vi "Abstract LV Class - Hierarchy.vi"   [LabVIEW 2021]
uses:
  Type/Abs_Type.lvclass
  Value/Abs_Value.lvclass
  Numeric/Abs_Numeric.lvclass
  Floating Point/Abs_Floating Point.lvclass
  Single Float/Abs_Single Float.lvclass
  Double Float/Abs_Double Float.lvclass
  Extended Float/Abs_Extended Float.lvclass
  Complex Double Float/Abs_Complex Double Float.lvclass
  Complex Extended Float/Abs_Complex Extended Float.lvclass
  Complex Single Float/Abs_Complex Single Float.lvclass
  Integer/Abs_Integer.lvclass
  I8 Integer/Abs_I8 Integer.lvclass
  I16 Integer/Abs_I16 Integer.lvclass
  I32 Integer/Abs_I32 Integer.lvclass
  I64 Integer/Abs_I64 Integer.lvclass
  U8 Integer/Abs_U8 Integer.lvclass
  U16 Integer/Abs_U16 Integer.lvclass
  U32 Integer/Abs_U32 Integer.lvclass
  U64 Integer/Abs_U64 Integer.lvclass
  Time/Abs_Time.lvclass
  Boolean/Abs_Boolean.lvclass
  String/Abs_String.lvclass
  Variant/Abs_Variant.lvclass
  Waveform/Abs_Waveform.lvclass
  Boolean/Static Write.vi
  Double Float/Simple Read.vi
  Boolean/Static Read.vi
panel:
  # "SEE DIAGRAM\nFOR Hierarchy"
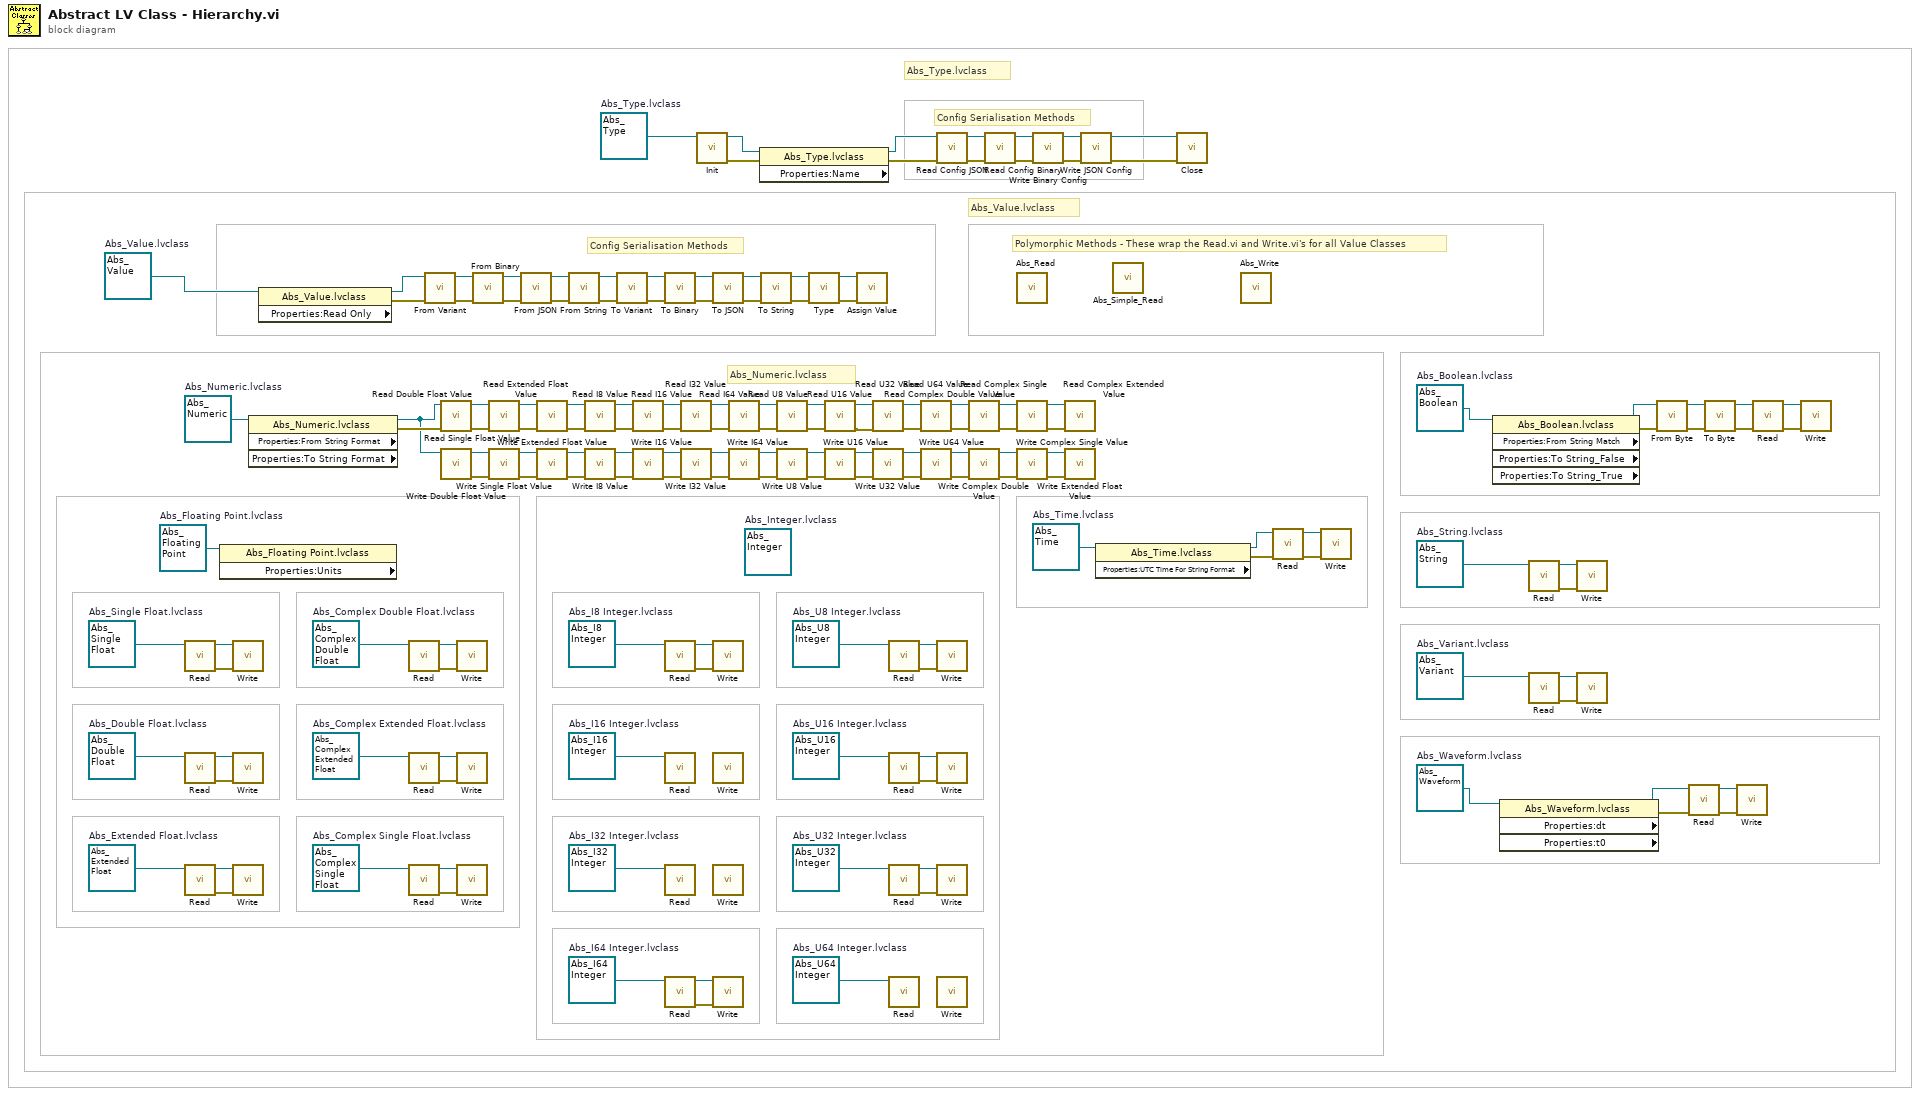
[diagram p0: block diagram]
diagram:
  w43 = refnum<class "Abs_Waveform.lvclass"> refnum  # Abs_Waveform.lvclass
  w44 = refnum<class "Abs_Variant.lvclass"> refnum  # Abs_Variant.lvclass
  w49 = refnum<class "Abs_String.lvclass"> refnum  # Abs_String.lvclass
  w58 = refnum<class "Abs_Boolean.lvclass"> refnum  # Abs_Boolean.lvclass
  w63 = refnum<class "Abs_Time.lvclass"> refnum  # Abs_Time.lvclass
  w73 = refnum<class "Abs_U64 Integer.lvclass"> refnum  # Abs_U64 Integer.lvclass
  w72 = refnum<class "Abs_U32 Integer.lvclass"> refnum  # Abs_U32 Integer.lvclass
  w70 = refnum<class "Abs_U16 Integer.lvclass"> refnum  # Abs_U16 Integer.lvclass
  w71 = refnum<class "Abs_U8 Integer.lvclass"> refnum  # Abs_U8 Integer.lvclass
  w76 = refnum<class "Abs_I64 Integer.lvclass"> refnum  # Abs_I64 Integer.lvclass
  w75 = refnum<class "Abs_I32 Integer.lvclass"> refnum  # Abs_I32 Integer.lvclass
  w74 = refnum<class "Abs_I16 Integer.lvclass"> refnum  # Abs_I16 Integer.lvclass
  w81 = refnum<class "Abs_I8 Integer.lvclass"> refnum  # Abs_I8 Integer.lvclass
  (unwired) refnum<class "Abs_Integer.lvclass"> refnum  # Abs_Integer.lvclass
  w84 = refnum<class "Abs_Complex Single Float.lvclass"> refnum  # Abs_Complex Single Float.lvclass
  w87 = refnum<class "Abs_Complex Extended Float.lvclass"> refnum  # Abs_Complex Extended Float.lvclass
  w90 = refnum<class "Abs_Complex Double Float.lvclass"> refnum  # Abs_Complex Double Float.lvclass
  w93 = refnum<class "Abs_Extended Float.lvclass"> refnum  # Abs_Extended Float.lvclass
  w96 = refnum<class "Abs_Double Float.lvclass"> refnum  # Abs_Double Float.lvclass
  w99 = refnum<class "Abs_Single Float.lvclass"> refnum  # Abs_Single Float.lvclass
  w100 = refnum<class "Abs_Floating Point.lvclass"> refnum  # Abs_Floating Point.lvclass
  w128 = refnum<class "Abs_Numeric.lvclass"> refnum  # Abs_Numeric.lvclass
  w38 = refnum<class "Abs_Value.lvclass"> refnum  # Abs_Value.lvclass
  w151 = refnum<class "Abs_Type.lvclass"> refnum  # Abs_Type.lvclass
  # "Abs_Numeric.lvclass"
  # "Polymorphic Methods - These wrap the Read.vi and Write.vi's for all Value Classes"
  # "Config Serialisation Methods"
  # "Abs_Value.lvclass"
  # "Abs_Type.lvclass"
  # "Config Serialisation Methods"
  n1 = call-dynamic "Read.vi"("Double Float.lvclass_340760 in"=w99) -> ("error out"=w97:errorcluster, "Double Float.lvclass_340760 out"=w98:refnum<class "Abs_Single Float.lvclass">)  [unwired: 8 in, 1 out]
  n2 = call-dynamic "Read.vi"("Double Float.lvclass_340760 in"=w96) -> ("error out"=w94:errorcluster, "Double Float.lvclass_340760 out"=w95:refnum<class "Abs_Double Float.lvclass">)  [unwired: 8 in, 1 out]
  n3 = call-dynamic "Read.vi"("Double Float.lvclass_340760 in"=w93) -> ("error out"=w91:errorcluster, "Double Float.lvclass_340760 out"=w92:refnum<class "Abs_Extended Float.lvclass">)  [unwired: 8 in, 1 out]
  n4 = property class="Abs_Floating Point.lvclass" props=["Properties:Units"](reference=w100) -> ()  [unwired: 1 in, 3 out]
  n5 = call-dynamic "Write.vi"("error in (no error)"=w97, "Double Float.lvclass_340760 in"=w98) -> ()  [unwired: 8 in, 2 out]
  n6 = call-dynamic "Write.vi"("error in (no error)"=w94, "Double Float.lvclass in"=w95) -> ()  [unwired: 8 in, 2 out]
  n7 = call-dynamic "Write.vi"("error in (no error)"=w91, "Double Float.lvclass_340760 in"=w92) -> ()  [unwired: 8 in, 2 out]
  n8 = property class="Abs_Numeric.lvclass" props=["Properties:From String Format", "Properties:To String Format"](reference=w128) -> (reference out=w29:refnum<class "Abs_Numeric.lvclass">, error out=w127:errorcluster)  [unwired: 1 in, 2 out]
  n9 = property class="Abs_Value.lvclass" props=["Properties:Read Only"](reference=w38) -> (reference out=w36:refnum<class "Abs_Value.lvclass">, error out=w37:errorcluster)  [unwired: 1 in, 1 out]
  n10 = call-dynamic "Read.vi"("Double Float.lvclass_340760 in"=w90) -> ("error out"=w88:errorcluster, "Double Float.lvclass_340760 out"=w89:refnum<class "Abs_Complex Double Float.lvclass">)  [unwired: 8 in, 1 out]
  n11 = call-dynamic "Read.vi"("Double Float.lvclass_340760 in"=w87) -> ("error out"=w85:errorcluster, "Double Float.lvclass_340760 out"=w86:refnum<class "Abs_Complex Extended Float.lvclass">)  [unwired: 8 in, 1 out]
  n12 = call-dynamic "Read.vi"("Double Float.lvclass_340760 in"=w84) -> ("error out"=w82:errorcluster, "Double Float.lvclass_340760 out"=w83:refnum<class "Abs_Complex Single Float.lvclass">)  [unwired: 8 in, 1 out]
  n13 = call-dynamic "From Variant.vi"("error in (no error)"=w37, "Abs_Value in"=w36) -> ("error out"=w34:errorcluster, "Abs_Value out"=w35:refnum<class "Abs_Value.lvclass">)  [unwired: 8 in]
  n14 = call-dynamic "Read Double Float Value.vi"("error in (no error)"=w127, "Numeric in"=w29) -> ("error out"=w117:errorcluster, "Numeric out"=w126:refnum<class "Abs_Numeric.lvclass">)  [unwired: 7 in, 1 out]
  n15 = call-dynamic "Write Double Float Value.vi"("Numeric in"=w29) -> ("error out"=w15:errorcluster, "Numeric out"=w28:refnum<class "Abs_Numeric.lvclass">)  [unwired: 9 in]
  n16 = call-dynamic "Write.vi"("error in (no error)"=w88, "Double Float.lvclass_340760 in"=w89) -> ()  [unwired: 8 in, 2 out]
  n17 = call-dynamic "Write.vi"("error in (no error)"=w85, "Double Float.lvclass_340760 in"=w86) -> ()  [unwired: 8 in, 2 out]
  n18 = call-dynamic "Write.vi"("error in (no error)"=w82, "Double Float.lvclass_340760 in"=w83) -> ()  [unwired: 8 in, 2 out]
  n19 = call-dynamic "From Binary.vi"("error in (no error)"=w34, "Type in"=w35) -> ("error out"=w133:errorcluster, "Type out"=w138:refnum<class "Abs_Value.lvclass">)  [unwired: 7 in, 1 out]
  n20 = call-dynamic "Read Single Float Value.vi"("error in (no error)"=w117, "Numeric in"=w126) -> ("error out"=w116:errorcluster, "Numeric out"=w125:refnum<class "Abs_Numeric.lvclass">)  [unwired: 7 in, 1 out]
  n21 = call-dynamic "Write Single Float Value.vi"("error in (no error)"=w15, "Numeric in"=w28) -> ("error out"=w14:errorcluster, "Numeric out"=w27:refnum<class "Abs_Numeric.lvclass">)  [unwired: 8 in]
  n22 = call-dynamic "From JSON.vi"("error in (no error)"=w133, "Type in"=w138) -> ("error out"=w132:errorcluster, "Type out"=w137:refnum<class "Abs_Value.lvclass">)  [unwired: 8 in]
  n23 = call-dynamic "Read Extended Float Value.vi"("error in (no error)"=w116, "Numeric in"=w125) -> ("error out"=w115:errorcluster, "Numeric out"=w124:refnum<class "Abs_Numeric.lvclass">)  [unwired: 7 in, 1 out]
  n24 = call-dynamic "Write Extended Float Value.vi"("error in (no error)"=w14, "Numeric in"=w27) -> ("error out"=w13:errorcluster, "Numeric out"=w26:refnum<class "Abs_Numeric.lvclass">)  [unwired: 8 in]
  n25 = call-dynamic "From String.vi"("error in (no error)"=w132, "Type in"=w137) -> ("error out"=w32:errorcluster, "Type out"=w33:refnum<class "Abs_Value.lvclass">)  [unwired: 6 in, 2 out]
  n26 = call-dynamic "Read I8 Value.vi"("error in (no error)"=w115, "Numeric in"=w124) -> ("error out"=w114:errorcluster, "Numeric out"=w123:refnum<class "Abs_Numeric.lvclass">)  [unwired: 7 in, 1 out]
  n27 = call-dynamic "Write I8 Value.vi"("error in (no error)"=w13, "Numeric in"=w26) -> ("error out"=w12:errorcluster, "Numeric out"=w25:refnum<class "Abs_Numeric.lvclass">)  [unwired: 8 in]
  n28 = call-dynamic "To Variant.vi"("error in (no error)"=w32, "Abs_Value in"=w33) -> ("error out"=w30:errorcluster, "Abs_Value out"=w31:refnum<class "Abs_Value.lvclass">)  [unwired: 7 in, 1 out]
  n29 = call-dynamic "Read I16 Value.vi"("error in (no error)"=w114, "Numeric in"=w123) -> ("error out"=w113:errorcluster, "Numeric out"=w122:refnum<class "Abs_Numeric.lvclass">)  [unwired: 7 in, 1 out]
  n30 = call-dynamic "Write I16 Value.vi"("error in (no error)"=w12, "Numeric in"=w25) -> ("error out"=w11:errorcluster, "Numeric out"=w24:refnum<class "Abs_Numeric.lvclass">)  [unwired: 8 in]
  n31 = call-dynamic "To Binary.vi"("error in (no error)"=w30, "Type in"=w31) -> ("error out"=w131:errorcluster, "Type out"=w136:refnum<class "Abs_Value.lvclass">)  [unwired: 7 in, 1 out]
  n32 = call-dynamic "Read.vi"("Double Float.lvclass_340760 in"=w81) -> ("error out"=w79:errorcluster, "Double Float.lvclass_340760 out"=w80:refnum<class "Abs_I8 Integer.lvclass">)  [unwired: 8 in, 1 out]
  n33 = call-dynamic "Read.vi"("Double Float.lvclass_340760 in"=w74) -> ()  [unwired: 8 in, 3 out]
  n34 = call-dynamic "Read.vi"("Double Float.lvclass_340760 in"=w75) -> ()  [unwired: 8 in, 3 out]
  n35 = call-dynamic "Read.vi"("Double Float.lvclass_340760 in"=w76) -> ("error out"=w77:errorcluster, "Double Float.lvclass_340760 out"=w78:refnum<class "Abs_I64 Integer.lvclass">)  [unwired: 8 in, 1 out]
  n36 = call-dynamic "Read I32 Value.vi"("error in (no error)"=w113, "Numeric in"=w122) -> ("error out"=w112:errorcluster, "Numeric out"=w121:refnum<class "Abs_Numeric.lvclass">)  [unwired: 7 in, 1 out]
  n37 = call-dynamic "Write I32 Value.vi"("error in (no error)"=w11, "Numeric in"=w24) -> ("error out"=w10:errorcluster, "Numeric out"=w23:refnum<class "Abs_Numeric.lvclass">)  [unwired: 8 in]
  n38 = call-dynamic "Init.vi"("Data in"=w151) -> ("error out"=w150:errorcluster, "Data out"=w149:refnum<class "Abs_Type.lvclass">)  [unwired: 9 in]
  n39 = call-dynamic "To JSON.vi"("error in (no error)"=w131, "Type in"=w136) -> ("error out"=w130:errorcluster, "Type out"=w135:refnum<class "Abs_Value.lvclass">)  [unwired: 7 in, 1 out]
  n40 = call-dynamic "Write.vi"("error in (no error)"=w79, "Double Float.lvclass_340760 in"=w80) -> ()  [unwired: 8 in, 2 out]
  n41 = call-dynamic "Write.vi"() -> ()  [unwired: 10 in, 2 out]
  n42 = call-dynamic "Write.vi"() -> ()  [unwired: 10 in, 2 out]
  n43 = call-dynamic "Write.vi"("error in (no error)"=w77, "Double Float.lvclass_340760 in"=w78) -> ()  [unwired: 8 in, 2 out]
  n44 = call-dynamic "Read I64 Value.vi"("error in (no error)"=w112, "Numeric in"=w121) -> ("error out"=w111:errorcluster, "Numeric out"=w120:refnum<class "Abs_Numeric.lvclass">)  [unwired: 7 in, 1 out]
  n45 = call-dynamic "Write I64 Value.vi"("error in (no error)"=w10, "Numeric in"=w23) -> ("error out"=w9:errorcluster, "Numeric out"=w22:refnum<class "Abs_Numeric.lvclass">)  [unwired: 8 in]
  n46 = property class="Abs_Type.lvclass" props=["Properties:Name"](reference=w149, error in=w150) -> (reference out=w147:refnum<class "Abs_Type.lvclass">, error out=w148:errorcluster)  [unwired: 1 out]
  n47 = call-dynamic "To String.vi"("error in (no error)"=w130, "Types in"=w135) -> ("error out"=w129:errorcluster, "Types out"=w134:refnum<class "Abs_Value.lvclass">)  [unwired: 7 in, 1 out]
  n48 = call-dynamic "Read U8 Value.vi"("error in (no error)"=w111, "Numeric in"=w120) -> ("error out"=w110:errorcluster, "Numeric out"=w119:refnum<class "Abs_Numeric.lvclass">)  [unwired: 7 in, 1 out]
  n49 = call-dynamic "Write U8 Value.vi"("error in (no error)"=w9, "Numeric in"=w22) -> ("error out"=w8:errorcluster, "Numeric out"=w21:refnum<class "Abs_Numeric.lvclass">)  [unwired: 8 in]
  n50 = call-dynamic "Type.vi"("error in (no error)"=w129, "Element in"=w134) -> ("error out"=w1:errorcluster, "Element out"=w2:refnum<class "Abs_Value.lvclass">)  [unwired: 7 in, 1 out]
  n51 = call-dynamic "Read U16 Value.vi"("error in (no error)"=w110, "Numeric in"=w119) -> ("error out"=w109:errorcluster, "Numeric out"=w118:refnum<class "Abs_Numeric.lvclass">)  [unwired: 7 in, 1 out]
  n52 = call-dynamic "Write U16 Value.vi"("error in (no error)"=w8, "Numeric in"=w21) -> ("error out"=w7:errorcluster, "Numeric out"=w20:refnum<class "Abs_Numeric.lvclass">)  [unwired: 8 in]
  n53 = call-dynamic "Assign Value.vi"("error in (no error)"=w1, "Abs_Value in"=w2) -> ()  [unwired: 8 in, 2 out]
  n54 = call-dynamic "Read U32 Value.vi"("error in (no error)"=w109, "Numeric in"=w118) -> ("error out"=w108:errorcluster, "Numeric out"=w107:refnum<class "Abs_Numeric.lvclass">)  [unwired: 7 in, 1 out]
  n55 = call-dynamic "Write U32 Value.vi"("error in (no error)"=w7, "Numeric in"=w20) -> ("error out"=w6:errorcluster, "Numeric out"=w19:refnum<class "Abs_Numeric.lvclass">)  [unwired: 8 in]
  n56 = call-dynamic "Read.vi"("Double Float.lvclass_340760 in"=w71) -> ("error out"=w68:errorcluster, "Double Float.lvclass_340760 out"=w69:refnum<class "Abs_U8 Integer.lvclass">)  [unwired: 8 in, 1 out]
  n57 = call-dynamic "Read.vi"("Double Float.lvclass_340760 in"=w70) -> ("error out"=w66:errorcluster, "Double Float.lvclass_340760 out"=w67:refnum<class "Abs_U16 Integer.lvclass">)  [unwired: 8 in, 1 out]
  n58 = call-dynamic "Read.vi"("Double Float.lvclass_340760 in"=w72) -> ("error out"=w64:errorcluster, "Double Float.lvclass_340760 out"=w65:refnum<class "Abs_U32 Integer.lvclass">)  [unwired: 8 in, 1 out]
  n59 = call-dynamic "Read.vi"("Double Float.lvclass_340760 in"=w73) -> ()  [unwired: 8 in, 3 out]
  n60 = call-dynamic "Read U64 Value.vi"("error in (no error)"=w108, "Numeric in"=w107) -> ("error out"=w105:errorcluster, "Numeric out"=w106:refnum<class "Abs_Numeric.lvclass">)  [unwired: 7 in, 1 out]
  n61 = call-dynamic "Write U64 Value.vi"("error in (no error)"=w6, "Numeric in"=w19) -> ("error out"=w5:errorcluster, "Numeric out"=w18:refnum<class "Abs_Numeric.lvclass">)  [unwired: 8 in]
  n62 = call "Read Config JSON.vi"("error in (no error)"=w148, "Abs_Type in"=w147) -> ("error out"=w146:errorcluster, "Abs_Type out"=w145:refnum<class "Abs_Type.lvclass">)  [unwired: 8 in]
  n63 = call-dynamic "Write.vi"("error in (no error)"=w68, "Double Float.lvclass_340760 in"=w69) -> ()  [unwired: 8 in, 2 out]
  n64 = call-dynamic "Write.vi"("error in (no error)"=w66, "Double Float.lvclass_340760 in"=w67) -> ()  [unwired: 8 in, 2 out]
  n65 = call-dynamic "Write.vi"("error in (no error)"=w64, "Double Float.lvclass_340760 in"=w65) -> ()  [unwired: 8 in, 2 out]
  n66 = call-dynamic "Write.vi"() -> ()  [unwired: 10 in, 2 out]
  n67 = call-dynamic "Read Complex Double Value.vi"("error in (no error)"=w105, "Numeric in"=w106) -> ("error out"=w104:errorcluster, "Numeric out"=w103:refnum<class "Abs_Numeric.lvclass">)  [unwired: 7 in, 1 out]
  n68 = call-dynamic "Write Complex Double Value.vi"("error in (no error)"=w5, "Numeric in"=w18) -> ("error out"=w4:errorcluster, "Numeric out"=w17:refnum<class "Abs_Numeric.lvclass">)  [unwired: 8 in]
  n69 = call "Read Config Binary.vi"("error in (no error)"=w146, "Abs_Type in"=w145) -> ("error out"=w144:errorcluster, "Abs_Type out"=w143:refnum<class "Abs_Type.lvclass">)  [unwired: 7 in, 1 out]
  n70 = call-poly "Abs_Read.vi"() -> ()  [unwired: 9 in, 3 out]
  n71 = call-dynamic "Read Complex Single Value.vi"("error in (no error)"=w104, "Numeric in"=w103) -> ("error out"=w101:errorcluster, "Numeric out"=w102:refnum<class "Abs_Numeric.lvclass">)  [unwired: 7 in, 1 out]
  n72 = call-dynamic "Write Complex Single Value.vi"("error in (no error)"=w4, "Numeric in"=w17) -> ("error out"=w3:errorcluster, "Numeric out"=w16:refnum<class "Abs_Numeric.lvclass">)  [unwired: 8 in]
  n73 = call-dynamic "Write Binary Config.vi"("error in (no error)"=w144, "Abs_Type in"=w143) -> ("error out"=w141:errorcluster, "Abs_Type out"=w142:refnum<class "Abs_Type.lvclass">)  [unwired: 7 in, 1 out]
  n74 = call-dynamic "Read Complex Extended Value.vi"("error in (no error)"=w101, "Numeric in"=w102) -> ()  [unwired: 7 in, 3 out]
  n75 = call-dynamic "Write Extended Float Value.vi"("error in (no error)"=w3, "Numeric in"=w16) -> ()  [unwired: 8 in, 2 out]
  n76 = call-dynamic "Write JSON Config.vi"("error in (no error)"=w141, "Abs_Type in"=w142) -> ("error out"=w140:errorcluster, "Abs_Type out"=w139:refnum<class "Abs_Type.lvclass">)  [unwired: 7 in, 1 out]
  n77 = property class="Abs_Time.lvclass" props=["Properties:UTC Time For String Format"](reference=w63) -> (reference out=w59:refnum<class "Abs_Time.lvclass">, error out=w62:errorcluster)  [unwired: 1 in, 1 out]
  n78 = call-poly "Abs_Simple_Read.vi"() -> ()  [unwired: 5 in, 1 out]
  n79 = call-dynamic "Close.vi"("error in (no error)"=w140, "Data in"=w139) -> ()  [unwired: 8 in, 2 out]
  n80 = call-poly "Abs_Write.vi"() -> ()  [unwired: 10 in, 2 out]
  n81 = call-dynamic "Read.vi"("error in (no error)"=w62, "Double Float.lvclass_340760 in"=w59) -> ("error out"=w61:errorcluster, "Double Float.lvclass_340760 out"=w60:refnum<class "Abs_Time.lvclass">)  [unwired: 7 in, 1 out]
  n82 = call-dynamic "Write.vi"("error in (no error)"=w61, "Double Float.lvclass_340760 in"=w60) -> ()  [unwired: 8 in, 2 out]
  n83 = property class="Abs_Boolean.lvclass" props=["Properties:From String Match", "Properties:To String_False", "Properties:To String_True"](reference=w58) -> (reference out=w56:refnum<class "Abs_Boolean.lvclass">, error out=w57:errorcluster)  [unwired: 1 in, 3 out]
  n84 = property class="Abs_Waveform.lvclass" props=["Properties:dt", "Properties:t0"](reference=w43) -> (reference out=w42:refnum<class "Abs_Waveform.lvclass">, error out=w41:errorcluster)  [unwired: 1 in, 2 out]
  n85 = call-dynamic "Read.vi"("Abs_String in"=w49) -> ("error out"=w47:errorcluster, "Abs_String out"=w48:refnum<class "Abs_String.lvclass">)  [unwired: 8 in, 1 out]
  n86 = call-dynamic "Read.vi"("Abs_Variant in"=w44) -> ("error out"=w45:errorcluster, "Abs_Variant out"=w46:refnum<class "Abs_Variant.lvclass">)  [unwired: 8 in, 1 out]
  n87 = call-dynamic "Write.vi"("error in (no error)"=w47, "Abs_String in"=w48) -> ()  [unwired: 8 in, 2 out]
  n88 = call-dynamic "Write.vi"("error in (no error)"=w45, "Abs_Variant in"=w46) -> ()  [unwired: 8 in, 2 out]
  n89 = call-dynamic "From Byte.vi"("error in (no error)"=w57, "Boolean in"=w56) -> ("error out"=w54:errorcluster, "Boolean out"=w55:refnum<class "Abs_Boolean.lvclass">)  [unwired: 8 in]
  n90 = call-dynamic "Read.vi"("error in (no error)"=w41, "Abs_Waveform in"=w42) -> ("error out"=w40:errorcluster, "Abs_Waveform out"=w39:refnum<class "Abs_Waveform.lvclass">)  [unwired: 7 in, 1 out]
  n91 = call-dynamic "To Byte.vi"("error in (no error)"=w54, "Boolean in"=w55) -> ("error out"=w52:errorcluster, "Boolean out"=w53:refnum<class "Abs_Boolean.lvclass">)  [unwired: 8 in]
  n92 = call-dynamic "Write.vi"("error in (no error)"=w40, "Abs_Waveform in"=w39) -> ()  [unwired: 8 in, 2 out]
  n93 = call-dynamic "Read.vi"("error in (no error)"=w52, "Boolean in"=w53) -> ("error out"=w50:errorcluster, "Boolean out"=w51:refnum<class "Abs_Boolean.lvclass">)  [unwired: 7 in, 1 out]
  n94 = call-dynamic "Write.vi"("error in (no error)"=w50, "Boolean in"=w51) -> ()  [unwired: 8 in, 2 out]
